vi "并列执行.vi"() -> ()   [LabVIEW 2021]
doc: "本VI是为《我和LabVIEW》一书编写的示例。\n关于本书的介绍请参考网页：\nhttp://ruanqizhen.spaces.live.com/blog/cns!5852D4F797C53FB6!4310.entry"
panel:
  out "error out":errorcluster
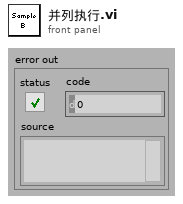
[diagram p1: front panel]
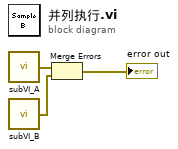
[diagram p0: block diagram]
diagram:
  n1 = call "subVI_A.vi"() -> ("error out"=w2:errorcluster)  [unwired: 1 in]
  n2 = call "subVI_B.vi"() -> ("error out"=w3:errorcluster)  [unwired: 1 in]
  n3 = Merge Errors "Merge Errors"(w2, w3) -> (→"error out":errorcluster)
